vi "Query Current Angle.vi"(8 "error in (no error)":errorcluster, 11 "AUDIX EM1000 in":refnum<class "AUDIX EM1000.lvclass">) -> (0 "error out":errorcluster, 2 "Current Angle":dbl, 3 "AUDIX EM1000 out":refnum<class "AUDIX EM1000.lvclass">)   [LabVIEW 2023, in "Turn Table and Mast.lvlib" / "AUDIX EM1000.lvclass"]
uses:
  AUDIX EM1000.lvclass
  AUDIX EM1000.lvclass/AUDIX EM1000.ctl
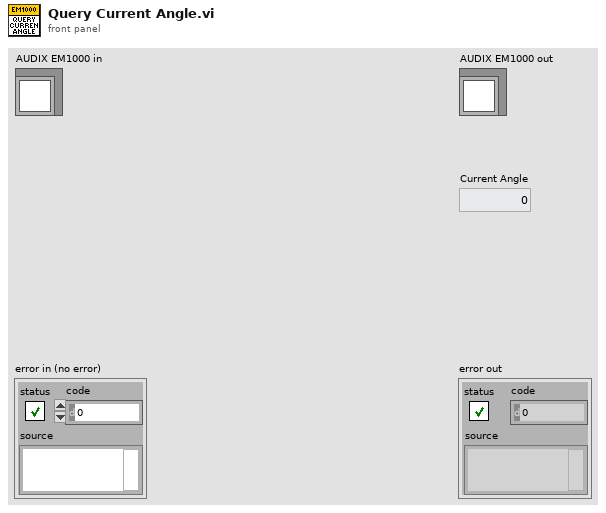
[diagram p1: front panel]
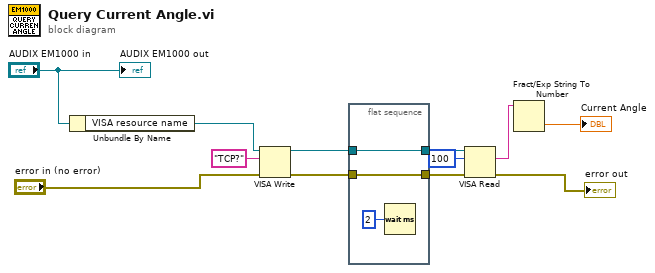
[diagram p0: block diagram]
diagram:
  n1 = Unbundle By Name("AUDIX EM1000 in") -> ("VISA resource name"=w9:refnum<visa-resource-name>)
  n2 = VISA Write(VISA resource name=w9, write buffer="TCP?" ("버퍼 쓰기"), error in (no error)="error in (no error)") -> (VISA resource name out=w5:refnum<visa-resource-name>, error out=w4:errorcluster)  [unwired: 1 out]
  n3 = flat-sequence {
    tunnel: w5 -> [w14]
    tunnel: w4 -> [w13]
    tunnel: [w14] -> w3
    tunnel: [w13] -> w2
    frame #0 {
      n4 = Wait (ms)(milliseconds to wait=u32 2) -> ()  [unwired: 1 out]
    }
  }
  n5 = VISA Read(VISA resource name=w3, byte count=u32 100, error in (no error)=w2) -> (read buffer=w10:string, error out=→"error out":errorcluster)  [unwired: 2 out]
  n6 = Fract/Exp String To Number(string=w10) -> (number=→"Current Angle":dbl)  [unwired: 3 in, 1 out]
  "AUDIX EM1000 out" <- "AUDIX EM1000 in"
